vi "FX_Close.vi"(10 "error in (no error)":errorcluster, 11 "PLC Conn":refnum<visa-resource-name>) -> (3 "error out":errorcluster)   [LabVIEW 2018]
doc: "Use this template to build a VI to use as a subVI."
panel:
  # "說明：關閉通訊埠。有錯誤也會執行。"
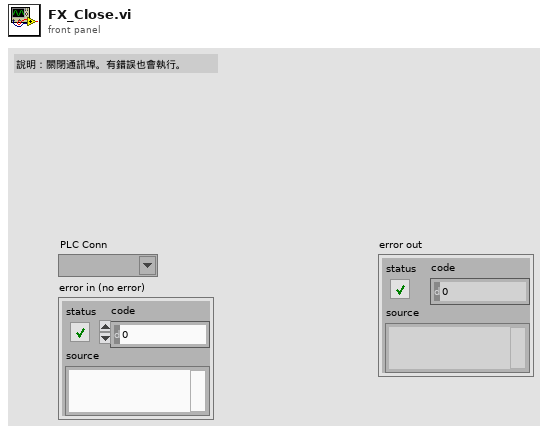
[diagram p1: front panel]
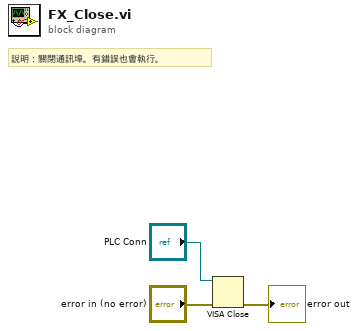
[diagram p0: block diagram]
diagram:
  # "說明：關閉通訊埠。有錯誤也會執行。"
  n1 = VISA Close(VISA resource name="PLC Conn", error in (no error)="error in (no error)") -> (error out=→"error out":errorcluster)
